vi "Uninstall Package.vi"(8 "error in":errorcluster, 11 "package name":string) -> (0 "error out":errorcluster, 3 "package name out":string)   [LabVIEW 2014, in "NIPM_API.lvlib"]
doc: "Uninstalls the specified package on this computer.\n\nNote: This VI will launch a Windows dialog asking for permission to run and requires the user to have admin rights.\n\nINPUT(s)\n<B>Package name</B>: Specifies the package to uninstall.\n\nOUTPUT(s)\n<B>Package name</B>: Outputs the requested package to uninstall."
uses:
  NIPM_API.lvlib
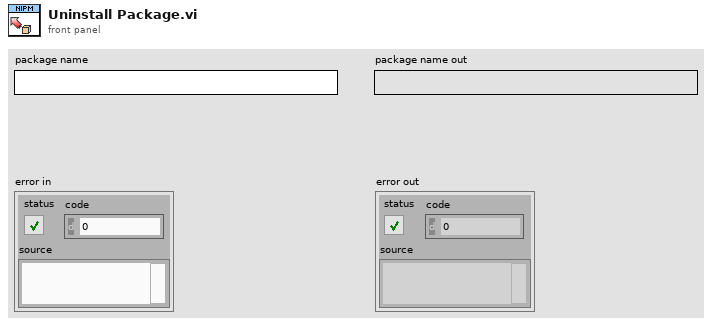
[diagram p1: front panel]
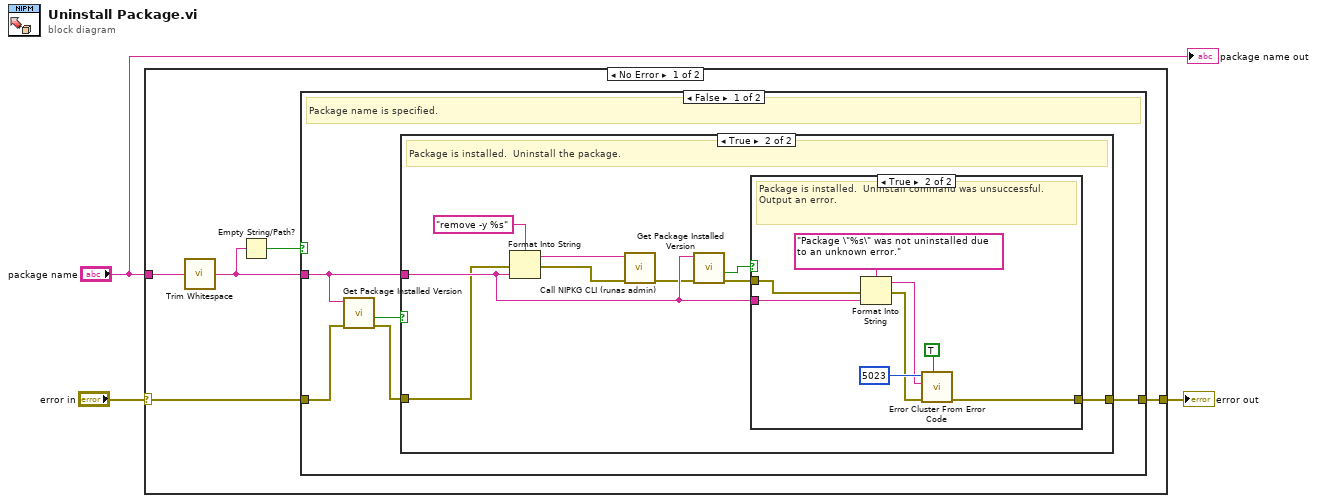
[diagram p0: block diagram]
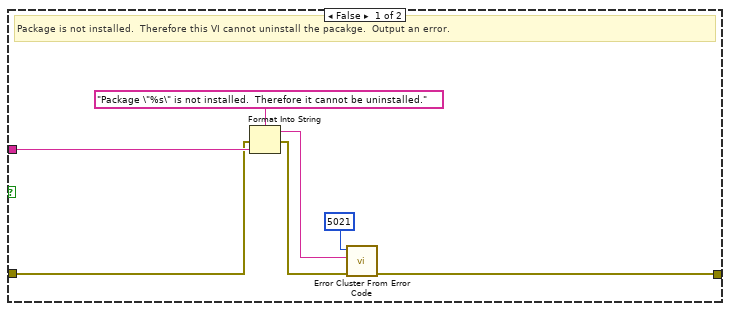
[diagram p2: hidden frame]
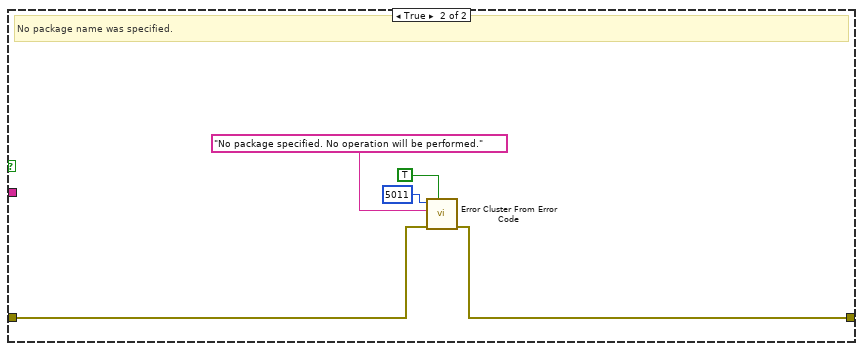
[diagram p4: hidden frame]
diagram:
  n1 = case shown="No Error" "error in" {
    selector: "error in" -> [w8 w44]
    tunnel: [w7 w44] -> w2
    tunnel: "package name" -> [w6 _]
    frame No Error {
      n2 = call <vilib>:"Trim Whitespace.vi"("string"=w6) -> ("trimmed string"=w5:string)  [unwired: 1 in]
      n3 = Empty String/Path?(string/path=w5) -> (empty?=w4:bool)
      n4 = case shown="False" w4 {
        tunnel: w8 -> [w11 w40]
        tunnel: [w13 w39] -> w7
        tunnel: w5 -> [w12 _]
        frame False {
          # "Package name is specified."
          n5 = call "Get Package Installed Version.vi"("error in"=w11, "package name"=w12) -> ("error out"=w9:errorcluster, "installed?"=w10:bool)  [unwired: 6 in, 2 out]
          n6 = case shown="True" w10 {
            tunnel: [w19 w26] -> w13
            tunnel: w12 -> [w17 w25]
            tunnel: w9 -> [w16 w24]
            frame False {
              # "Package is not installed.  Therefore this VI cannot uninstall the pacakge.  Output an error."
              n7 = Format Into String(format string="Package \"%s\" is not installed.  Therefore it cannot be uninstalled.", error in=w16, w17) -> (resulting string=w14:string, error out=w15:errorcluster)  [unwired: 1 in]
              n8 = call <vilib>:"Error Cluster From Error Code.vi"("error in (no error)"=w15, "error message (\"\")"=w14, "error code (0)"=5021) -> ("error out"=w19:errorcluster)  [unwired: 6 in]
            }
            frame True {
              # "Package is installed.  Uninstall the package."
              n9 = Format Into String(format string="remove -y %s", error in=w24, w25) -> (resulting string=w27:string, error out=w28:errorcluster)  [unwired: 1 in]
              n10 = call "Call NIPKG CLI (runas admin).vi"("error in (no error)"=w28, "command"=w27) -> ("error out"=w23:errorcluster)  [unwired: 9 in]
              n11 = call "Get Package Installed Version.vi"("error in"=w23, "package name"=w25) -> ("error out"=w21:errorcluster, "installed?"=w22:bool)  [unwired: 6 in, 2 out]
              n12 = case shown="True" w22 {
                tunnel: w21 -> [w30 w33]
                tunnel: [w30 w36] -> w26
                tunnel: w25 -> [_ w32]
                frame False {
                  # "Package is not installed.  Uninstall command was successful."
                }
                frame True {
                  # "Package is installed.  Uninstall command was unsuccessful.  Output an error."
                  n13 = Format Into String(format string="Package \"%s\" was not uninstalled due to an unknown error.", error in=w33, w32) -> (resulting string=w31:string, error out=w34:errorcluster)  [unwired: 1 in]
                  n14 = call <vilib>:"Error Cluster From Error Code.vi"("show call chain? (False)"=TRUE, "error in (no error)"=w34, "error message (\"\")"=w31, "error code (0)"=5023) -> ("error out"=w36:errorcluster)  [unwired: 5 in]
                }
              }
            }
          }
        }
        frame True {
          # "No package name was specified."
          n15 = call <vilib>:"Error Cluster From Error Code.vi"("show call chain? (False)"=TRUE, "error in (no error)"=w40, "error message (\"\")"="No package specified. No operation will be performed.", "error code (0)"=5011) -> ("error out"=w39:errorcluster)  [unwired: 5 in]
        }
      }
    }
    frame Error {
    }
  }
  "error out" <- w2
  "package name out" <- "package name"
